vi "Stages Messenger.vi"(0 "Stage Notifier Name":string="ProScan3", 2 "Actions":T2, 5 "Setpoint":dbl[](array[numeric]), 7 "Axis":bool[](array[boolean]), 9 "Velocity":dbl, 11 "Misc":variant, 12 "Servo On?":bool, 13 "Exit While Busy?":bool) -> (4 "Stage Notifier Name (Dup)":string, 6 "Positions":dbl[](array[numeric]), 8 "Status":T1, 10 "Servo Status":bool, 15 "Error":errorcluster)   [LabVIEW 2021]
uses:
  Stages Controls/Stage Actions.ctl
  Stages Controls/Stage Status.ctl
  Stages Controls/Stage Notifier Element.ctl
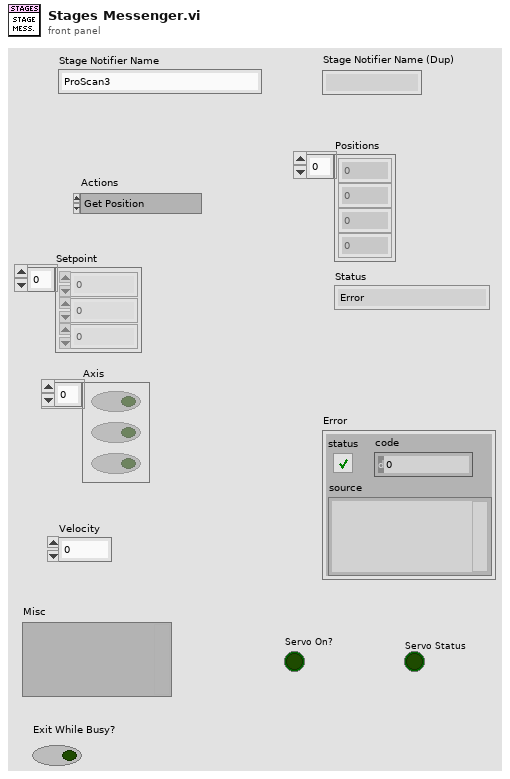
[diagram p1: front panel]
types:
  T1 = typedef "Stage Status.ctl" = enum16{"Error", "Abort", "Busy", "On Target"}
  T2 = typedef "Stage Actions.ctl" = enum16{"Get Position", "SERVO OFF", "SERVO ON", "SERVO ON/OFF", "MVR", "MOVE", "HALT", "ONTARGET", "ERROR", "REFERENCE", "INIT", "VELOCITY", "STATUS", "EXIT", "HOME", "ZEROPOS", "NANOPOS", "ANALOG", "QUIT"}
  T3 = typedef "Stage Notifier Element.ctl" = cluster{"Action":T2, "Axis":bool[], "Setpoint":dbl[], "Velocity":dbl, "Cmd Recvd?":bool, "Position":dbl[], "Status":T1, "Misc":variant, "Servo On?":bool}
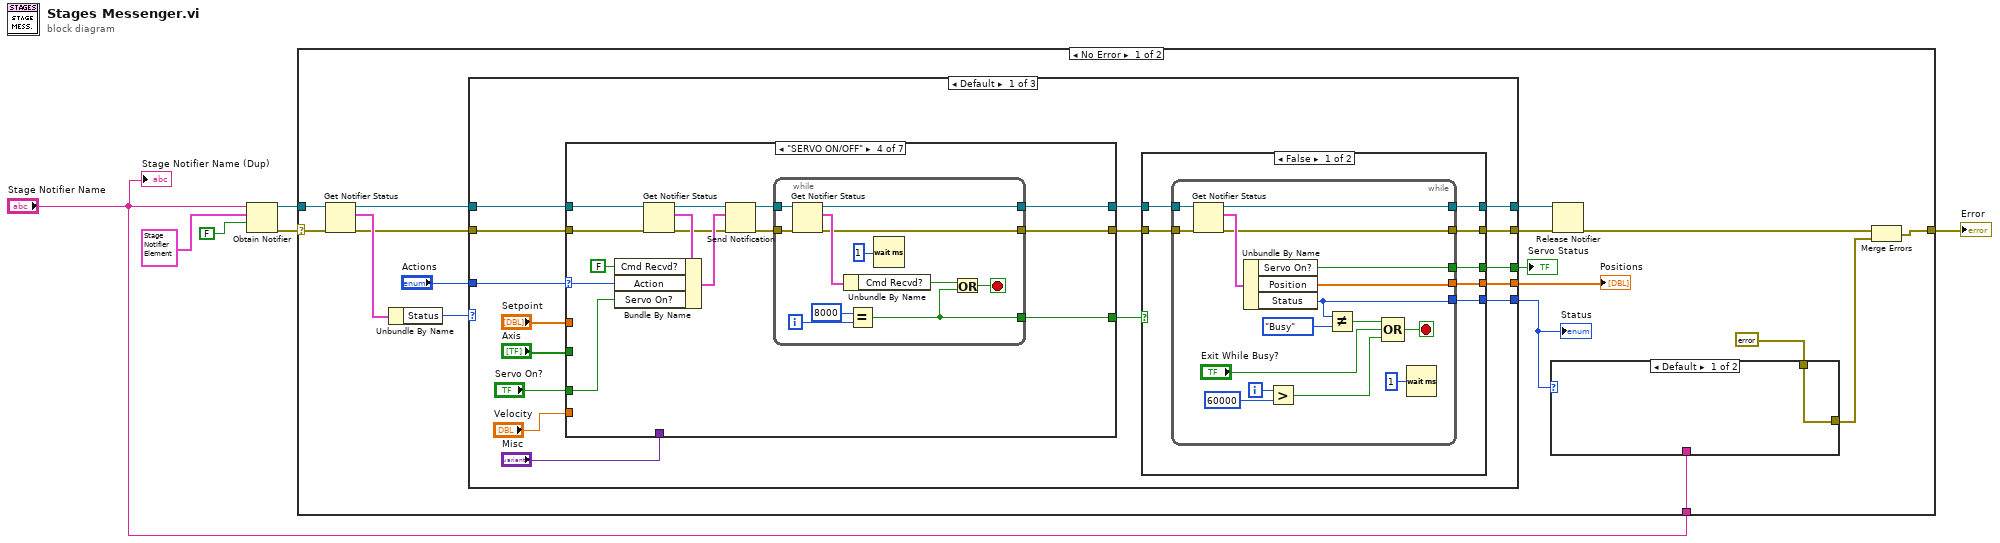
[diagram p0: block diagram]
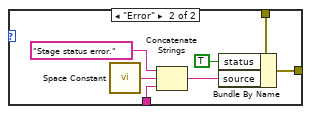
[diagram p2: hidden frame]
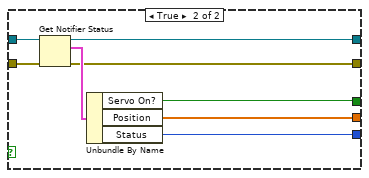
[diagram p3: hidden frame]
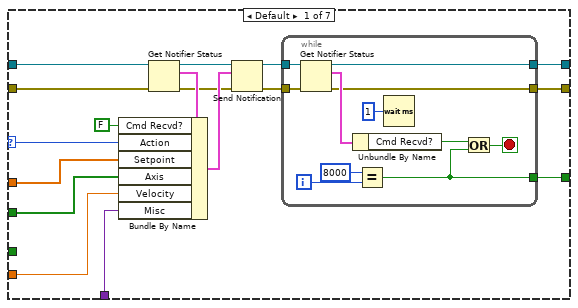
[diagram p4: hidden frame]
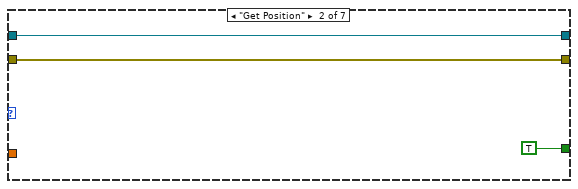
[diagram p5: hidden frame]
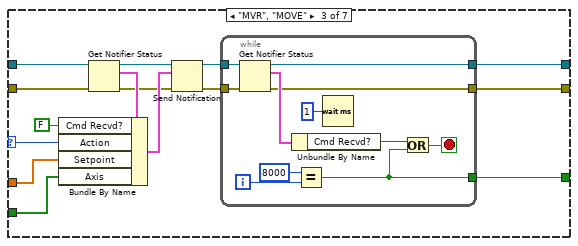
[diagram p6: hidden frame]
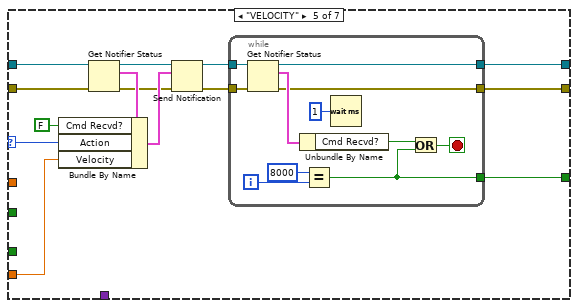
[diagram p7: hidden frame]
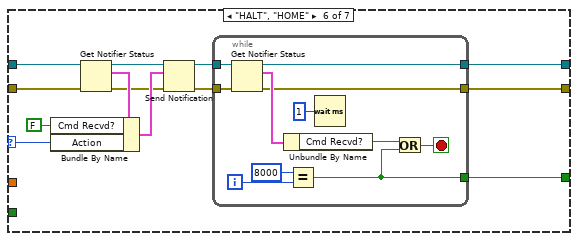
[diagram p8: hidden frame]
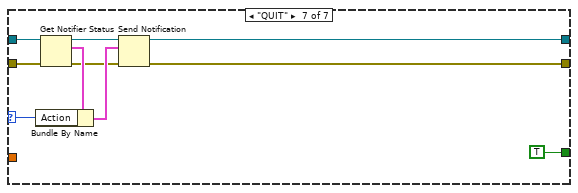
[diagram p9: hidden frame]
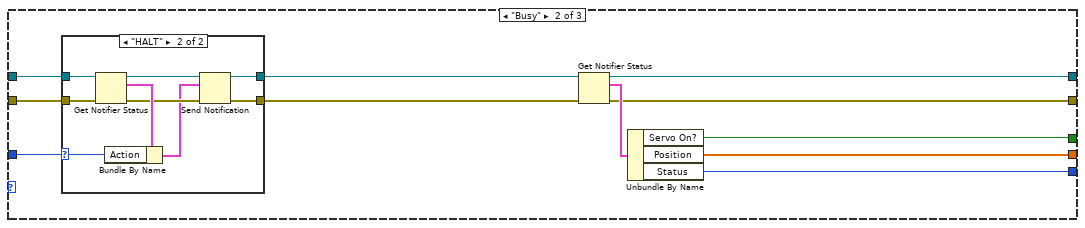
[diagram p10: hidden frame]
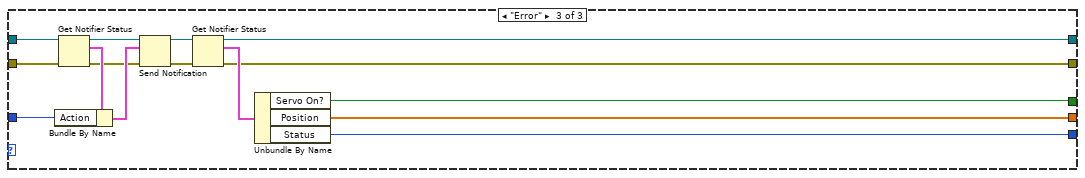
[diagram p12: hidden frame]
diagram:
  n1 = Obtain Notifier(name (unnamed)="Stage Notifier Name", notification data type=T3 {"Action"=enum."Get Position", "Axis"=[], "Setpoint"=[], "Velocity"=0.5, "Cmd Recvd?"=FALSE, "Position"=[], "Status"=enum."Error", "Misc"=variant, "Servo On?"=FALSE} ("Stage Status"), create if not found? (T)=FALSE) -> (notifier out=w3:refnum<notifier>, error out=w4:errorcluster)  [unwired: 1 in, 1 out]
  n2 = case shown="No Error" w4 {
    selector: w4 -> [w17 w257]
    tunnel: w3 -> [w23 _]
    tunnel: "Stage Notifier Name" -> [w12 _]
    tunnel: [w9 w257] -> w1
    frame No Error {
      n3 = Get Notifier Status(notifier=w23, error in (no error)=w17) -> (notifier out=w21:refnum<notifier>, current notification=w22:T3, error out=w16:errorcluster)  [unwired: 2 out]
      n4 = Unbundle By Name(w22) -> ("Status"=w14:T1)
      n5 = case shown="Default" w14 {
        tunnel: w21 -> [w47 w224 w256]
        tunnel: [w40 w229 w250] -> w20
        tunnel: [w39 w228 w249] -> w19
        tunnel: [w38 w227 w248] -> w13
        tunnel: "Actions" -> [w46 w225 w254]
        tunnel: w16 -> [w37 w223 w246]
        tunnel: [w35 w226 w243] -> w15
        tunnel: [w32 w220 w242] -> w7
        frame Default {
          n6 = case shown="\"SERVO ON/OFF\"" w46 {
            selector: w46 -> [w91 _ w120 w145 w170 w194 w215]
            tunnel: w47 -> [w92 w109 w121 w146 w171 w195 w218]
            tunnel: [w84 w109 w115 w142 w167 w191 w219] -> w41
            tunnel: "Setpoint" -> [w88 _ w117 _ _ _ _]
            tunnel: "Axis" -> [w87 _ w116 _ _ _ _]
            tunnel: "Velocity" -> [w86 _ _ _ w161 _ _]
            tunnel: "Misc" -> [w85 _ _ _ _ _ _]
            tunnel: [w83 TRUE w114 w141 w166 w190 TRUE] -> w42
            tunnel: w37 -> [w82 w108 w113 w140 w165 w189 w212]
            tunnel: [w79 w108 w110 w137 w162 w186 w210] -> w36
            tunnel: "Servo On?" -> [_ _ _ w136 _ _ _]
            frame Default {
              n7 = Get Notifier Status(notifier=w92, error in (no error)=w82) -> (notifier out=w93:refnum<notifier>, current notification=w94:T3, error out=w81:errorcluster)  [unwired: 2 out]
              n8 = Bundle By Name(cluster=w94, "Cmd Recvd?"=FALSE, "Action"=w91, "Setpoint"=w88, "Axis"=w87, "Velocity"=w86, "Misc"=w85) -> (w95:T3)
              n9 = Send Notification(notification=w95, notifier=w93, error in (no error)=w81) -> (notifier out=w89:refnum<notifier>, error out=w80:errorcluster)
              n10 = while {
                tunnel: w89 -> [w106]
                tunnel: [w103] -> w84
                tunnel: [w99] -> w83
                tunnel: w80 -> [w97]
                tunnel: [w96] -> w79
                i -> [w102]
                stop <- w98 stop-if-true
                n11 = Get Notifier Status(notifier=w106, error in (no error)=w97) -> (notifier out=w103:refnum<notifier>, current notification=w105:T3, error out=w96:errorcluster)  [unwired: 2 out]
                n12 = Unbundle By Name(w105) -> ("Cmd Recvd?"=w100:bool)
                n13 = Equal?(x=8000, y=w102) -> (x = y?=w99:bool)
                n14 = Wait (ms)(milliseconds to wait=u32 1) -> ()  [unwired: 1 out]
                n15 = Or(x=w100, y=w99) -> (x .or. y?=w98:bool)
              }
            }
            frame "Get Position" {
            }
            frame "MVR", "MOVE" {
              n16 = Get Notifier Status(notifier=w121, error in (no error)=w113) -> (notifier out=w122:refnum<notifier>, current notification=w123:T3, error out=w112:errorcluster)  [unwired: 2 out]
              n17 = Bundle By Name(cluster=w123, "Cmd Recvd?"=FALSE, "Action"=w120, "Setpoint"=w117, "Axis"=w116) -> (w124:T3)
              n18 = Send Notification(notification=w124, notifier=w122, error in (no error)=w112) -> (notifier out=w118:refnum<notifier>, error out=w111:errorcluster)
              n19 = while {
                tunnel: w118 -> [w135]
                tunnel: [w132] -> w115
                tunnel: [w128] -> w114
                tunnel: w111 -> [w126]
                tunnel: [w125] -> w110
                i -> [w131]
                stop <- w127 stop-if-true
                n20 = Get Notifier Status(notifier=w135, error in (no error)=w126) -> (notifier out=w132:refnum<notifier>, current notification=w134:T3, error out=w125:errorcluster)  [unwired: 2 out]
                n21 = Unbundle By Name(w134) -> ("Cmd Recvd?"=w129:bool)
                n22 = Equal?(x=8000, y=w131) -> (x = y?=w128:bool)
                n23 = Wait (ms)(milliseconds to wait=u32 1) -> ()  [unwired: 1 out]
                n24 = Or(x=w129, y=w128) -> (x .or. y?=w127:bool)
              }
            }
            frame "SERVO ON/OFF" {
              n25 = Get Notifier Status(notifier=w146, error in (no error)=w140) -> (notifier out=w147:refnum<notifier>, current notification=w148:T3, error out=w139:errorcluster)  [unwired: 2 out]
              n26 = Bundle By Name(cluster=w148, "Cmd Recvd?"=FALSE, "Action"=w145, "Servo On?"=w136) -> (w149:T3)
              n27 = Send Notification(notification=w149, notifier=w147, error in (no error)=w139) -> (notifier out=w143:refnum<notifier>, error out=w138:errorcluster)
              n28 = while {
                tunnel: w143 -> [w160]
                tunnel: [w157] -> w142
                tunnel: [w153] -> w141
                tunnel: w138 -> [w151]
                tunnel: [w150] -> w137
                i -> [w156]
                stop <- w152 stop-if-true
                n29 = Get Notifier Status(notifier=w160, error in (no error)=w151) -> (notifier out=w157:refnum<notifier>, current notification=w159:T3, error out=w150:errorcluster)  [unwired: 2 out]
                n30 = Unbundle By Name(w159) -> ("Cmd Recvd?"=w154:bool)
                n31 = Equal?(x=8000, y=w156) -> (x = y?=w153:bool)
                n32 = Wait (ms)(milliseconds to wait=u32 1) -> ()  [unwired: 1 out]
                n33 = Or(x=w154, y=w153) -> (x .or. y?=w152:bool)
              }
            }
            frame "VELOCITY" {
              n34 = Get Notifier Status(notifier=w171, error in (no error)=w165) -> (notifier out=w172:refnum<notifier>, current notification=w173:T3, error out=w164:errorcluster)  [unwired: 2 out]
              n35 = Bundle By Name(cluster=w173, "Cmd Recvd?"=FALSE, "Action"=w170, "Velocity"=w161) -> (w174:T3)
              n36 = Send Notification(notification=w174, notifier=w172, error in (no error)=w164) -> (notifier out=w168:refnum<notifier>, error out=w163:errorcluster)
              n37 = while {
                tunnel: w168 -> [w185]
                tunnel: [w182] -> w167
                tunnel: [w178] -> w166
                tunnel: w163 -> [w176]
                tunnel: [w175] -> w162
                i -> [w181]
                stop <- w177 stop-if-true
                n38 = Get Notifier Status(notifier=w185, error in (no error)=w176) -> (notifier out=w182:refnum<notifier>, current notification=w184:T3, error out=w175:errorcluster)  [unwired: 2 out]
                n39 = Unbundle By Name(w184) -> ("Cmd Recvd?"=w179:bool)
                n40 = Equal?(x=8000, y=w181) -> (x = y?=w178:bool)
                n41 = Wait (ms)(milliseconds to wait=u32 1) -> ()  [unwired: 1 out]
                n42 = Or(x=w179, y=w178) -> (x .or. y?=w177:bool)
              }
            }
            frame "HALT", "HOME" {
              n43 = Get Notifier Status(notifier=w195, error in (no error)=w189) -> (notifier out=w196:refnum<notifier>, current notification=w197:T3, error out=w188:errorcluster)  [unwired: 2 out]
              n44 = Bundle By Name(cluster=w197, "Cmd Recvd?"=FALSE, "Action"=w194) -> (w198:T3)
              n45 = Send Notification(notification=w198, notifier=w196, error in (no error)=w188) -> (notifier out=w192:refnum<notifier>, error out=w187:errorcluster)
              n46 = while {
                tunnel: w192 -> [w209]
                tunnel: [w206] -> w191
                tunnel: [w202] -> w190
                tunnel: w187 -> [w200]
                tunnel: [w199] -> w186
                i -> [w205]
                stop <- w201 stop-if-true
                n47 = Get Notifier Status(notifier=w209, error in (no error)=w200) -> (notifier out=w206:refnum<notifier>, current notification=w208:T3, error out=w199:errorcluster)  [unwired: 2 out]
                n48 = Unbundle By Name(w208) -> ("Cmd Recvd?"=w203:bool)
                n49 = Equal?(x=8000, y=w205) -> (x = y?=w202:bool)
                n50 = Wait (ms)(milliseconds to wait=u32 1) -> ()  [unwired: 1 out]
                n51 = Or(x=w203, y=w202) -> (x .or. y?=w201:bool)
              }
            }
            frame "QUIT" {
              n52 = Get Notifier Status(notifier=w218, error in (no error)=w212) -> (notifier out=w217:refnum<notifier>, current notification=w216:T3, error out=w211:errorcluster)  [unwired: 2 out]
              n53 = Bundle By Name(cluster=w216, "Action"=w215) -> (w214:T3)
              n54 = Send Notification(notification=w214, notifier=w217, error in (no error)=w211) -> (notifier out=w219:refnum<notifier>, error out=w210:errorcluster)
            }
          }
          n55 = case shown="False" w42 {
            tunnel: w41 -> [w54 w78]
            tunnel: [w53 w77] -> w40
            tunnel: [w52 w76] -> w39
            tunnel: [w51 w74] -> w38
            tunnel: w36 -> [w50 w73]
            tunnel: [w49 w72] -> w35
            tunnel: [w48 w71] -> w32
            frame False {
              n56 = while {
                tunnel: w54 -> [w70]
                tunnel: [w69] -> w53
                tunnel: [w67] -> w52
                tunnel: [w61] -> w51
                tunnel: w50 -> [w57]
                tunnel: [w56] -> w49
                tunnel: [w55] -> w48
                i -> [w63]
                stop <- w58 stop-if-true
                n57 = Get Notifier Status(notifier=w70, error in (no error)=w57) -> (notifier out=w69:refnum<notifier>, current notification=w68:T3, error out=w56:errorcluster)  [unwired: 2 out]
                n58 = Unbundle By Name(w68) -> ("Servo On?"=w55:bool, "Position"=w67:dbl[], "Status"=w61:T1)
                n59 = Greater?(x=w63, y=60000) -> (0:w59:bool)
                n60 = Not Equal?(x=w61, y=Stage_Status."Busy") -> (x != y?=w64:bool)
                n61 = Compound Arithmetic op=OR(w64, "Exit While Busy?", w59) -> (w58:bool)
                n62 = Wait (ms)(milliseconds to wait=u32 1) -> ()  [unwired: 1 out]
              }
            }
            frame True {
              n63 = Get Notifier Status(notifier=w78, error in (no error)=w73) -> (notifier out=w77:refnum<notifier>, current notification=w75:T3, error out=w72:errorcluster)  [unwired: 2 out]
              n64 = Unbundle By Name(w75) -> ("Servo On?"=w71:bool, "Position"=w76:dbl[], "Status"=w74:T1)
            }
          }
        }
        frame "Busy" {
          n65 = case shown="\"HALT\"" w225 {
            selector: w225 -> [_ w238]
            tunnel: w224 -> [w232 w241]
            tunnel: w223 -> [w231 w240]
            tunnel: [w232 w235] -> w222
            tunnel: [w231 w234] -> w221
            frame Default {
            }
            frame "HALT" {
              n66 = Get Notifier Status(notifier=w241, error in (no error)=w240) -> (notifier out=w237:refnum<notifier>, current notification=w239:T3, error out=w236:errorcluster)  [unwired: 2 out]
              n67 = Bundle By Name(cluster=w239, "Action"=w238) -> (w233:T3)
              n68 = Send Notification(notification=w233, notifier=w237, error in (no error)=w236) -> (notifier out=w235:refnum<notifier>, error out=w234:errorcluster)
            }
          }
          n69 = Get Notifier Status(notifier=w222, error in (no error)=w221) -> (notifier out=w229:refnum<notifier>, current notification=w230:T3, error out=w226:errorcluster)  [unwired: 2 out]
          n70 = Unbundle By Name(w230) -> ("Servo On?"=w220:bool, "Position"=w228:dbl[], "Status"=w227:T1)
        }
        frame "Error" {
          n71 = Get Notifier Status(notifier=w256, error in (no error)=w246) -> (notifier out=w253:refnum<notifier>, current notification=w255:T3, error out=w245:errorcluster)  [unwired: 2 out]
          n72 = Bundle By Name(cluster=w255, "Action"=w254) -> (w252:T3)
          n73 = Send Notification(notification=w252, notifier=w253, error in (no error)=w245) -> (notifier out=w251:refnum<notifier>, error out=w244:errorcluster)
          n74 = Get Notifier Status(notifier=w251, error in (no error)=w244) -> (notifier out=w250:refnum<notifier>, current notification=w247:T3, error out=w243:errorcluster)  [unwired: 2 out]
          n75 = Unbundle By Name(w247) -> ("Servo On?"=w242:bool, "Position"=w249:dbl[], "Status"=w248:T1)
        }
      }
      "Positions" <- w19
      "Status" <- w13
      "Servo Status" <- w7
      n76 = case shown="Default" w13 {
        tunnel: w12 -> [_ w28]
        tunnel: [w24 w26] -> w10
        tunnel: errorcluster {"status"=FALSE, "code"=0, "source"=""} ("Error 2") -> [w24 w25]
        frame Default {
        }
        frame "Error" {
          n77 = call <vilib>:"Space Constant.vi"() -> ("String"=w29:string)
          n78 = Concatenate Strings("Stage status error." ("source"), w29, w28) -> (w27:string)
          n79 = Bundle By Name(cluster=w25, "status"=TRUE, "source"=w27) -> (w26:errorcluster)
        }
      }
      n80 = Release Notifier(notifier=w20, error in (no error)=w15) -> (error out=w11:errorcluster)  [unwired: 1 in, 2 out]
      n81 = Merge Errors(w11, w10) -> (w9:errorcluster)
    }
    frame Error {
    }
  }
  "Error" <- w1
  "Stage Notifier Name (Dup)" <- "Stage Notifier Name"
